vi "File Exists.vi"   [LabVIEW 2020, in "openg_file.lvlib"]
doc: "Checks to see whether a path exists on disk and whether it is a directory."
uses:
  openg_file.lvlib
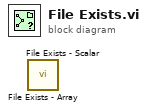
[diagram p0: block diagram]
diagram:
  n1 = call "File Exists - Array.vi"() -> ()  [unwired: 7 in, 2 out]
  n2 = call "File Exists - Scalar.vi"() -> ()  [unwired: 7 in, 2 out]
